vi "Select Black Level.vi"(8 "error in (no error)":errorcluster, 10 "Black Level Selection":string, 11 "Camera in":refnum<class "Camera.lvclass">) -> (0 "error out":errorcluster, 3 "Camera":refnum<class "Camera.lvclass">)   [LabVIEW 2020, in "Camera.lvclass"]
uses:
  Camera.lvclass
  Camera.lvclass/Camera.ctl
  bin/gindustrialcam_32-1.dll
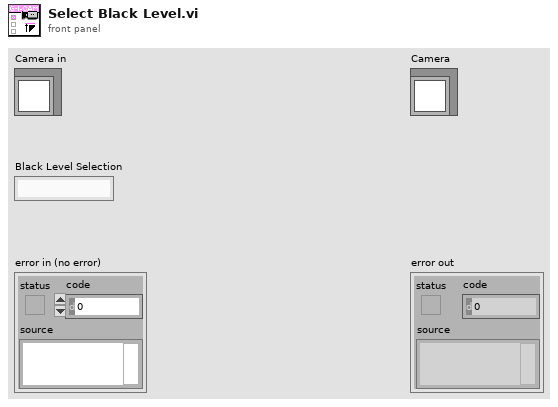
[diagram p1: front panel]
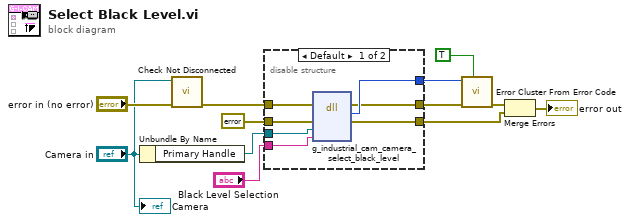
[diagram p0: block diagram]
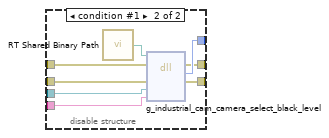
[diagram p2: hidden frame]
diagram:
  n1 = Unbundle By Name("Camera in") -> ("Primary Handle"=w8:refnum<data-value>)
  n2 = call "Check Not Disconnected.vi"("error in (no error)"="error in (no error)", "Camera in"="Camera in") -> ("error out"=w7:errorcluster)  [unwired: 9 in]
  n3 = disable-structure shown="Default" {
    disable-tunnel: "Black Level Selection" -> [w19 w27]
    disable-tunnel: w8 -> [w18 w26]
    disable-tunnel: w7 -> [w17 w25]
    disable-tunnel: errorcluster {"status"=FALSE, "code"=0, "source"=""} ("error constant") -> [w16 w24]
    disable-tunnel: [w15 w23] -> w4
    disable-tunnel: [w14 w22] -> w2
    disable-tunnel: [w13 w21] -> w1
    frame condition #0 (active) {
      n4 = dll-call lib="C:/serenial/lib/g-industrial-camera/LabVIEW/g_industrial_cam/bin/gindustrialcam_*-1.*" fn="g_industrial_cam_camera_select_black_level"(error in=w17, "err"=w16, "edvr"=w18, "formats"=w19) -> (error out=w13:errorcluster, "Mg_Error"=w14:i32, "err"=w15:errorcluster)  [unwired: 4 in, 1 out]
    }
    frame condition #1 {
      n5 = call "RT Shared Binary Path.vi"() -> ("Path"=w20:path)
      n6 = dll-call lib="C:/serenial/lib/g-industrial-camera/LabVIEW/g_industrial_cam/bin/gindustrialcam_*-1.*" fn="g_industrial_cam_camera_select_black_level"(path in=w20, error in=w25, "err"=w24, "edvr"=w26, "formats"=w27) -> (error out=w21:errorcluster, "Mg_Error"=w22:i32, "err"=w23:errorcluster)  [unwired: 3 in, 1 out]
    }
  }
  n7 = call <vilib>:"Error Cluster From Error Code.vi"("show call chain? (False)"=TRUE, "error in (no error)"=w1, "error code (0)"=w2) -> ("error out"=w3:errorcluster)  [unwired: 6 in]
  n8 = Merge Errors(w3, w4) -> (→"error out":errorcluster)
  "Camera" <- "Camera in"
